vi "RT_Actuator_Adapter.vi"(8 "error in (no error)":errorcluster={"status"=FALSE, "code"=0, "source"="\"\""}, 10 "permission":string, 11 "Logical actuator command":string) -> (0 "error out":errorcluster={"status"=FALSE, "code"=0, "source"="\"\""}, 2 "status ok":bool, 3 "Applied ACK/status":string)   [LabVIEW 2026]
doc: "INTENT: Control other rig actuators. LOGIC: Map logical ON/OFF/position commands to validated I/O channels; include readback."
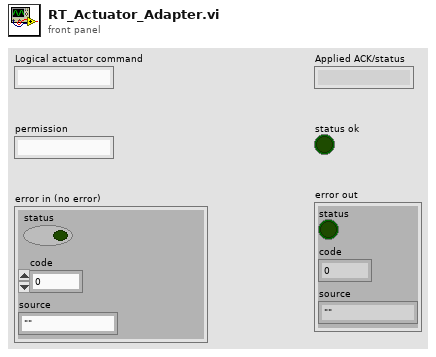
[diagram p1: front panel]
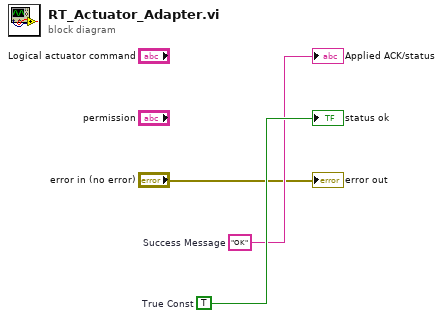
[diagram p0: block diagram]
diagram:
  w3 = TRUE  # True Const
  w2 = "OK"  # Success Message
  "Applied ACK/status" <- w2
  "status ok" <- w3
  "error out" <- "error in (no error)"
